vi "scale.vi"(0 "reference":refnum<class "Graphics.lvclass">, 1 "scaleX":dbl=1.0 format="%.2f", 2 "scaleY":dbl=1.0 format="%.2f", 5 "error in (no error)":errorcluster) -> (14 "reference out":refnum<class "Graphics.lvclass">, 19 "error out":errorcluster)   [LabVIEW 2020, in "Graphics.lvclass"]
doc: "Scale (x,y)\n1 is default\nMust be bigger than 0"
uses:
  <resource>/Framework/Providers/Open_GDS/UML/Graphics_class/Graphics.lvclass
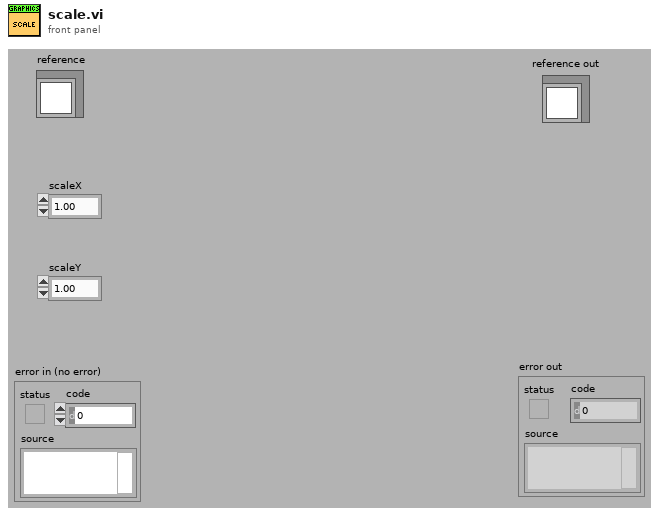
[diagram p1: front panel]
types:
  T1 = typedef "Graphics.lvclass/ObjectAttributes.ctl" = cluster{"drawColor":u32, "backgroundColor":u32, "font":T2, "fontType":T3, "picture":picture, "stroke":T4, "scaleX":dbl, "scaleY":dbl, "screenRef":refnum<vi>, "offsetX":dbl, "offsetY":dbl}
  T2 = typedef "Graphics.lvclass/FontType.ctl" = cluster{"Font Name:":string, "Size":i16, "Strikeout?":bool, "Italic?":bool, "Underline?":bool, "Outline?":bool, "Shadow?":bool, "Bold?":bool}
  T3 = typedef "Graphics.lvclass/LvFontType.ctl" = enum16{"User-specified Font", "Application Font", "System Font", "Dialog Font"}
  T4 = typedef "Graphics.lvclass/StrokeType.ctl" = enum16{"USE_DEFAULT", "SOLID", "DOTTED"}
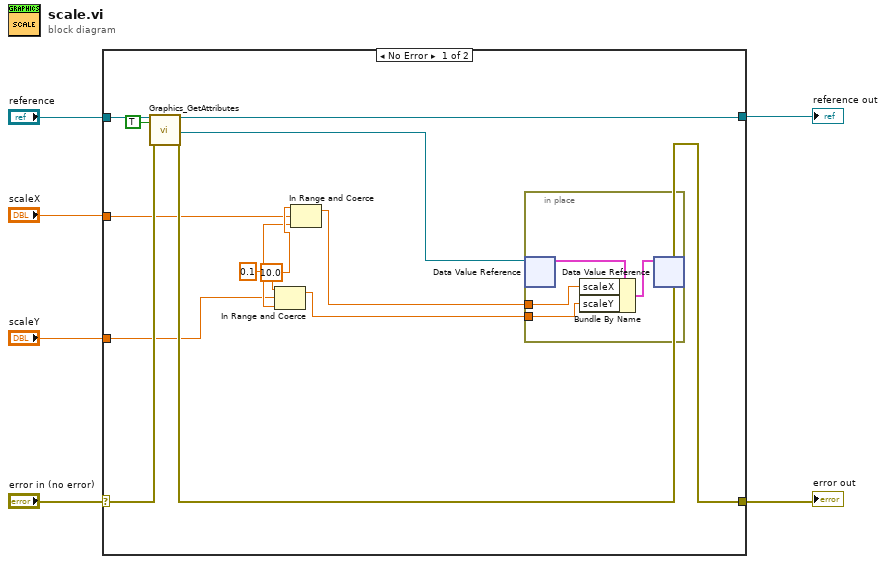
[diagram p0: block diagram]
diagram:
  n1 = case shown="No Error" "error in (no error)" {
    selector: "error in (no error)" -> [w18 w23]
    tunnel: "reference" -> [w17 w24]
    tunnel: [w16 w23] -> w4
    tunnel: [w15 w24] -> w3
    tunnel: "scaleX" -> [w12 _]
    tunnel: "scaleY" -> [w11 _]
    frame No Error {
      w14 = 10.0 ("upper limit")
      w13 = 0.1 ("lower limit")
      n2 = call <resource>:"Graphics_GetAttributes.vi"("reference in"=w17, "OnlyGetDvrReference(False)"=TRUE, "error in (no error)"=w18) -> ("reference out"=w15:refnum<class "Graphics.lvclass">, "DataRef"=w9:refnum<data-value>, "error out"=w16:errorcluster)  [unwired: 13 in, 1 out]
      n3 = In Range and Coerce(upper limit=w14, x=w11, lower limit=w13) -> (coerced(x)=w7:dbl)  [unwired: 1 out]
      n4 = In Range and Coerce(upper limit=w14, x=w12, lower limit=w13) -> (coerced(x)=w8:dbl)  [unwired: 1 out]
      n5 = in-place {
        in-place-border: w8 -> [w21]
        in-place-border: w7 -> [w20]
        n6 = in-place-dvr #1(w9) -> (w22:T1)  [unwired: 1 out]
        n7 = Bundle By Name(cluster=w22, "scaleX"=w21, "scaleY"=w20) -> (w19:T1)
        n8 = in-place-dvr #1(w19) -> ()  [unwired: 2 out]
      }
    }
    frame Error {
    }
  }
  "reference out" <- w3
  "error out" <- w4
